vi "Grab.vi"   [LabVIEW 2017]
uses:
  <vilib>/FPGAPlugInAG/myRIO-1900/niLvFpga_Open_myRIO-1900.vi
  <vilib>/rvi/interface/common/dynamic/niFpgaDynamicAddResources.vi
  <vilib>/Utility/error.llb/Error Cluster From Error Code.vi
  <vilib>/rvi/errors/niLvFpgaAdjustHostInterfaceError.vi
  <vilib>/FPGAPlugInAG/Dynamic/niLvFpga_Run_Dynamic.vi
  <vilib>/FPGAPlugInAG/Dynamic/niLvFpga_Close_Dynamic.vi
  <vilib>/rvi/interface/nirviOpenFPGA/nirviOpenFPGA.xnode
  FPGA Bitfiles/BadassLoader_FPGATarget_DCMotorControlle_4dRX-8eX8o0.lvbitx
  FPGA/DC Motor Controller (FPGA).vi
  <vilib>/rvi/interface/nirviReadWriteControl/nirviReadWriteControl.xnode
  <vilib>/rvi/interface/nirviMethod/nirviMethod.xnode
  <vilib>/rvi/interface/nirviCloseFPGA/nirviCloseFPGA.xnode
  <vilib>/rvi/interface/Simulation/niFpgaSimulationCallBeginRW.vi
  NiFpgaLv.dll
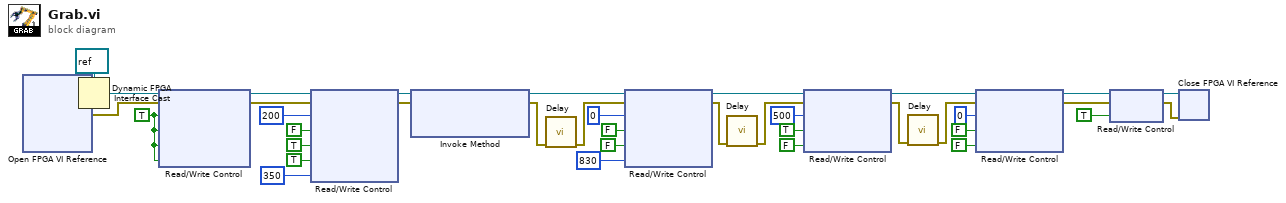
[diagram p0: block diagram]
diagram:
  w1 = TRUE ("DCmotor_0_A")
  n1 = xnode "Open FPGA VI Reference"() -> ("FPGA VI Reference Out"=w35:refnum<k20>, "error out"=w2:errorcluster)  [unwired: 2 in]
  n2 = Dynamic FPGA Interface Cast(Session In=refnum<k20> refnum ("FPGA Interface"), Type=w35) -> (Session Out=w5:refnum<k20>)
  n3 = xnode "Read/Write Control"("FPGA VI Reference In"=w5, "error in"=w2, "DCmotor_0_A"=w1, "DCmotor_0_B"=w1, "DCmotor_1_A"=w1, "DCmotor_1_B"=w1) -> ("FPGA VI Reference Out"=w4:refnum<k20>, "error out"=w3:errorcluster)
  n4 = xnode "Read/Write Control"("FPGA VI Reference In"=w4, "error in"=w3, "Motor Power"=u32 200, "M2_A"=FALSE, "M2_B"=TRUE, "S 6"=TRUE, "Servo 6"=u32 350) -> ("FPGA VI Reference Out"=w33:refnum<k20>, "error out"=w32:errorcluster)
  n5 = xnode "Invoke Method"("FPGA VI Reference In"=w33, "error in"=w32) -> ("FPGA VI Reference Out"=w25:refnum<k20>, "error out"=w27:errorcluster)  [unwired: 1 in]
  n6 = call "Delay"("error in (no error)"=w27) -> ("error out"=w24:errorcluster)  [unwired: 10 in]
  n7 = xnode "Read/Write Control"("FPGA VI Reference In"=w25, "error in"=w24, "Motor Power"=u32 0, "M2_A"=FALSE, "M2_B"=FALSE, "Servo 6"=u32 830) -> ("FPGA VI Reference Out"=w18:refnum<k20>, "error out"=w19:errorcluster)
  n8 = call "Delay"("error in (no error)"=w19) -> ("error out"=w17:errorcluster)  [unwired: 10 in]
  n9 = xnode "Read/Write Control"("FPGA VI Reference In"=w18, "error in"=w17, "Motor Power"=u32 500, "M2_A"=TRUE, "M2_B"=FALSE) -> ("FPGA VI Reference Out"=w12:refnum<k20>, "error out"=w13:errorcluster)
  n10 = call "Delay"("error in (no error)"=w13) -> ("error out"=w11:errorcluster)  [unwired: 10 in]
  n11 = xnode "Read/Write Control"("FPGA VI Reference In"=w12, "error in"=w11, "Motor Power"=u32 0, "M2_A"=FALSE, "M2_B"=FALSE) -> ("FPGA VI Reference Out"=w7:refnum<k20>, "error out"=w6:errorcluster)
  n12 = xnode "Read/Write Control"("FPGA VI Reference In"=w7, "error in"=w6, "stop"=TRUE) -> ("FPGA VI Reference Out"=w38:refnum<k20>, "error out"=w37:errorcluster)
  n13 = xnode "Close FPGA VI Reference"("FPGA VI Reference In"=w38, "error in"=w37) -> ()  [unwired: 1 out]
